vi "Test_Prepare_Checks_Caraya.vi"(8 "error in":errorcluster) -> (0 "error out":errorcluster)   [LabVIEW 2026]
doc: "Caraya tests of Prepare Checks: comparison text to enum, group contents kept, unknown comparison refused."
uses:
  <vilib>/addons/_JKI Toolkits/Caraya/classes/Test/Test.lvclass
  <vilib>/addons/_JKI Toolkits/Caraya/classes/Assert/Assert.lvclass
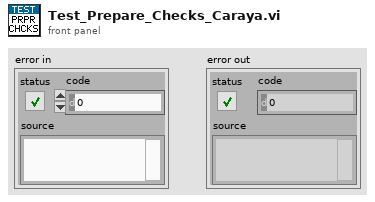
[diagram p1: front panel]
types:
  T1 = cluster{"di_high":cluster{"and":string[], "or":string[]}, "di_low":cluster{"and":string[], "or":string[]}, "misc_high":cluster{"and":string[], "or":string[]}, "misc_low":cluster{"and":string[], "or":string[]}, "t0_high":cluster{"and":cluster{"name":string, "min":dbl, "max":dbl}[], "or":cluster{"name":string, "min":dbl, "max":dbl}[]}, "t0_low":cluster{"and":cluster{"name":string, "min":dbl, "max":dbl}[], "or":cluster{"name":string, "min":dbl, "max":dbl}[]}, "misc_compare":cluster{"name":string, "compare_with":string, "comparison":string, "tolerance":dbl}[]}
  T2 = cluster{"di_high":cluster{"and_list":string[], "or_list":string[]}, "di_low":cluster{"and_list":string[], "or_list":string[]}, "misc_high":cluster{"and_list":string[], "or_list":string[]}, "misc_low":cluster{"and_list":string[], "or_list":string[]}, "t0_high":cluster{"and_list":cluster{"name":string, "min":dbl, "max":dbl}[], "or_list":cluster{"name":string, "min":dbl, "max":dbl}[]}, "t0_low":cluster{"and_list":cluster{"name":string, "min":dbl, "max":dbl}[], "or_list":cluster{"name":string, "min":dbl, "max":dbl}[]}, "misc_compare":cluster{"name":string, "compare_with":string, "comparison":enum16{"EQ", "NE", "GT", "GE", "LT", "LE"}, "tolerance":dbl}[]}
  T3 = cluster{"and_list":cluster{"name":string, "min":dbl, "max":dbl}[], "or_list":cluster{"name":string, "min":dbl, "max":dbl}[]}
  T4 = cluster{"name":string, "compare_with":string, "comparison":enum16{"EQ", "NE", "GT", "GE", "LT", "LE"}, "tolerance":dbl}[]
  T5 = cluster{"name":string, "compare_with":string, "comparison":enum16{"EQ", "NE", "GT", "GE", "LT", "LE"}, "tolerance":dbl}
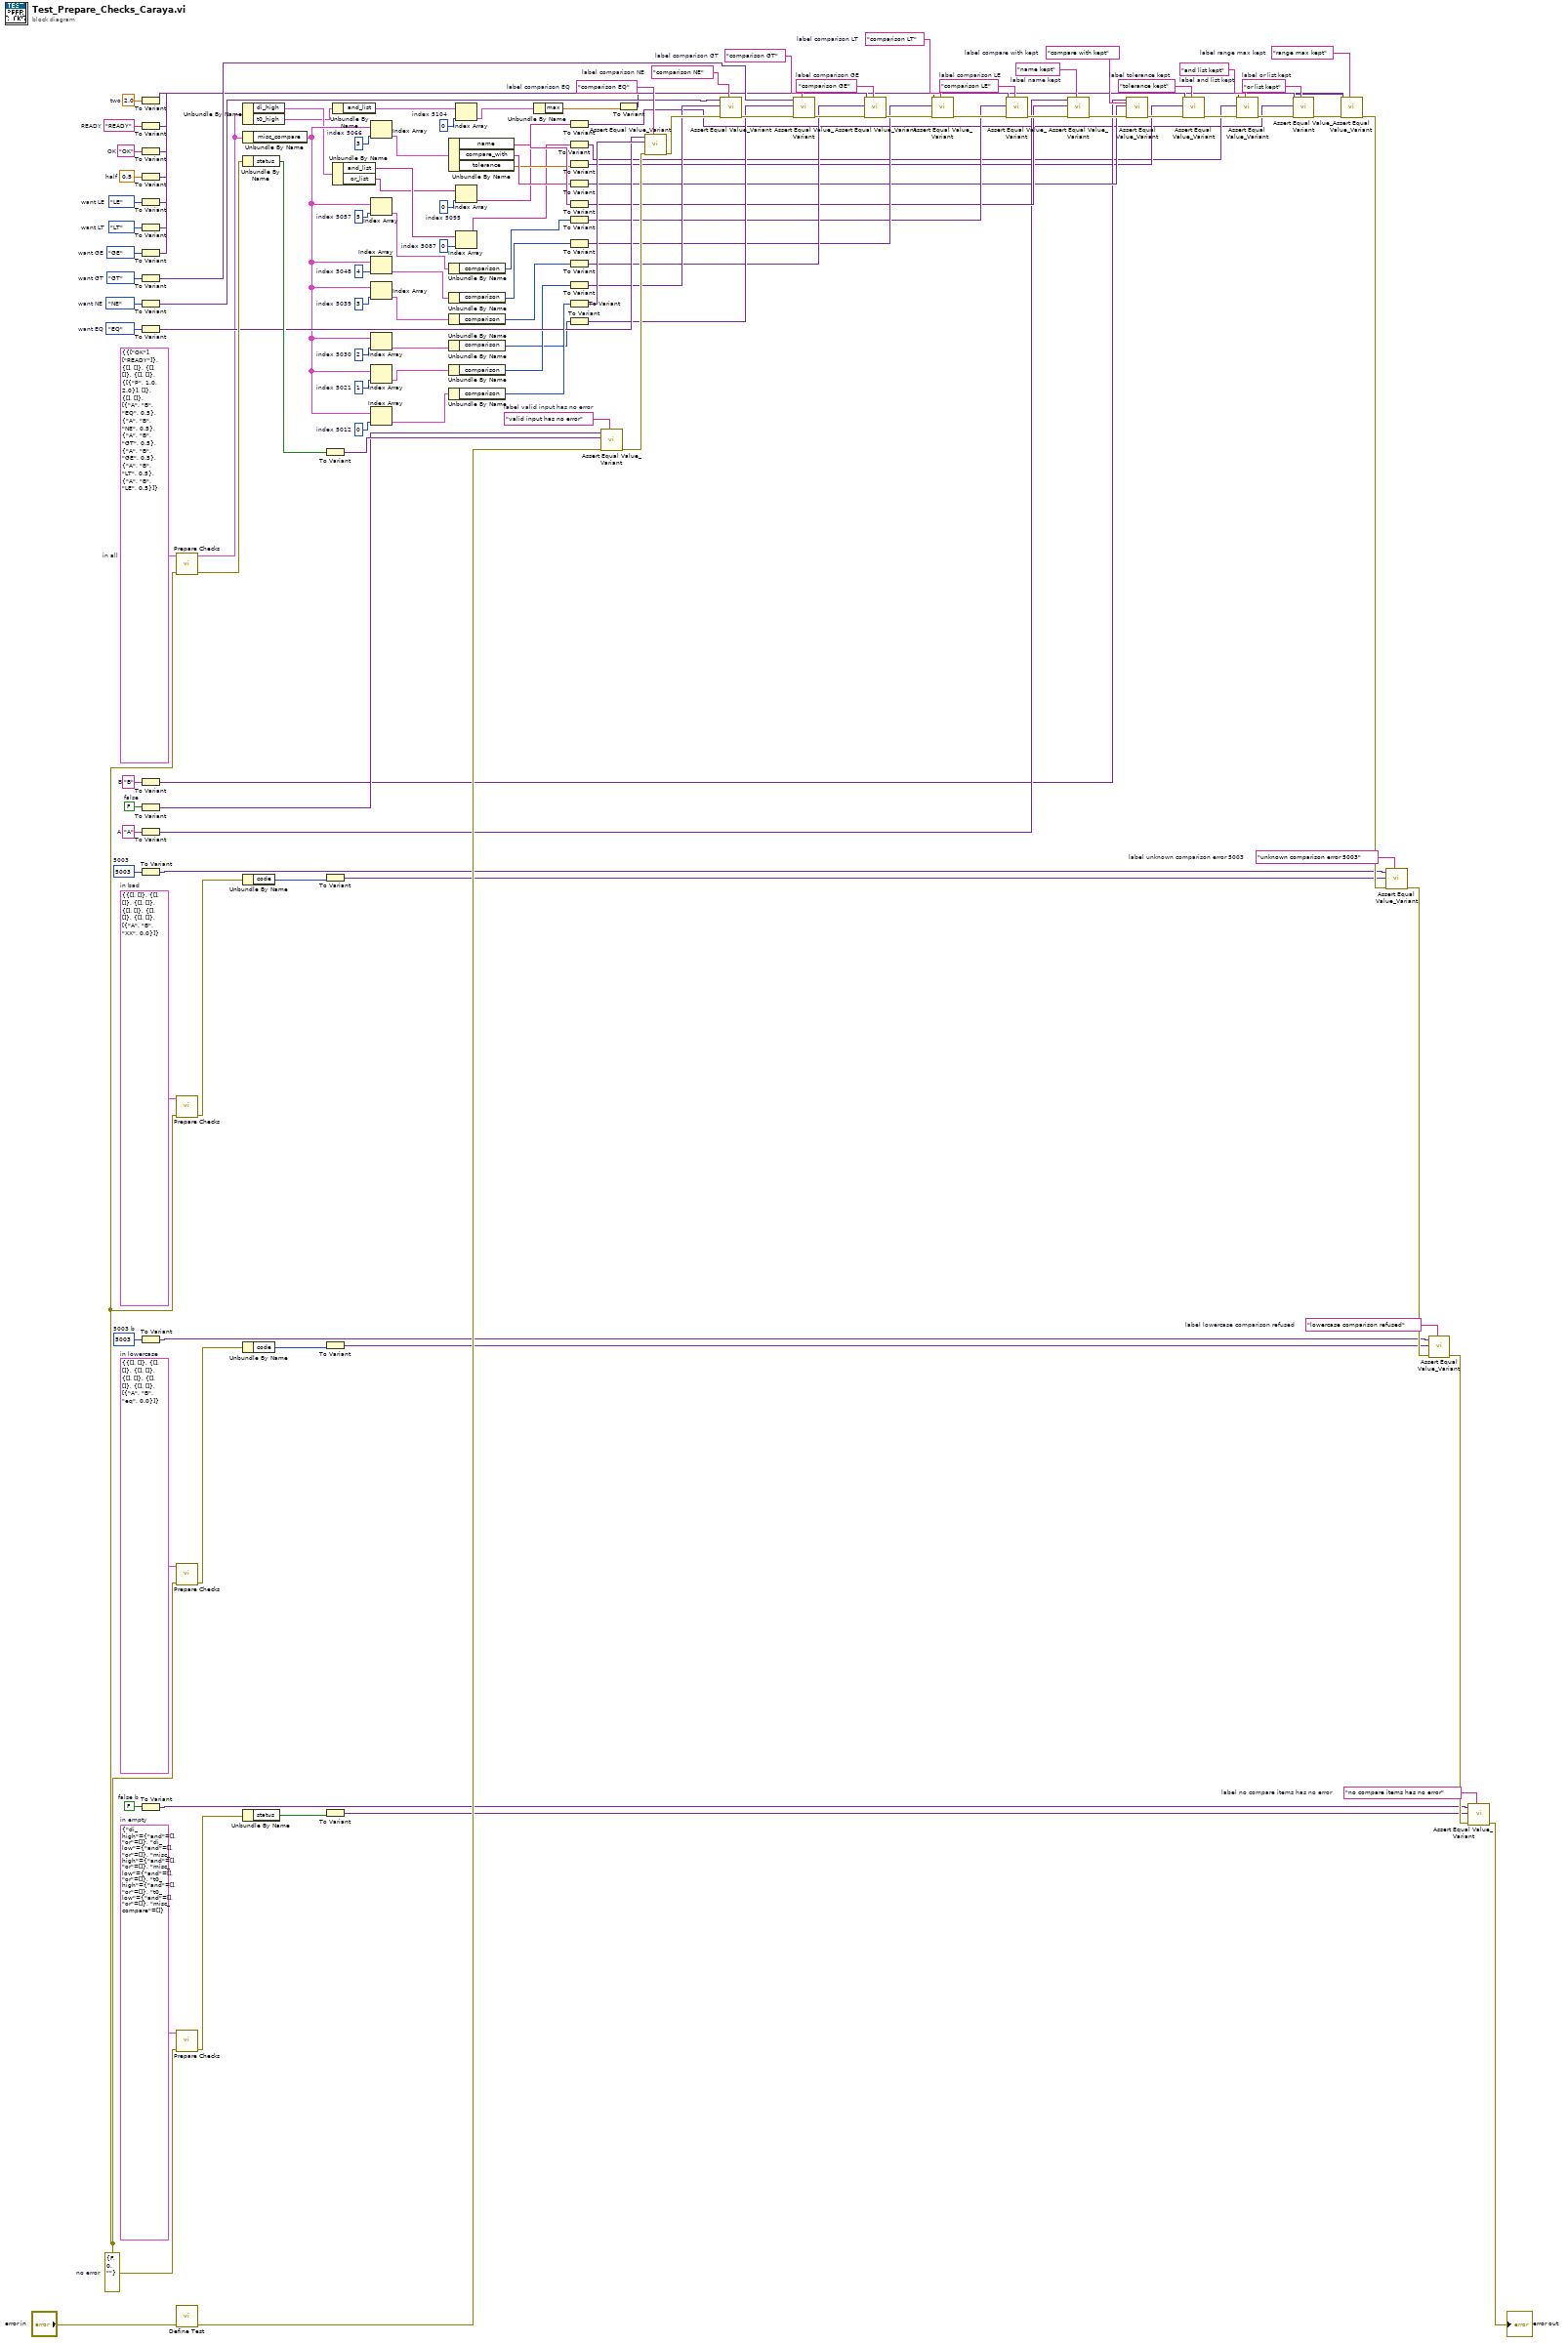
[diagram p0: block diagram]
diagram:
  w5 = "no compare items has no error"  # label no compare items has no error
  w6 = FALSE  # false b
  w10 = T1 {"di_high"={"and"=[], "or"=[]}, "di_low"={"and"=[], "or"=[]}, "misc_high"={"and"=[], "or"=[]}, "misc_low"={"and"=[], "or"=[]}, "t0_high"={"and"=[], "or"=[]}, "t0_low"={"and"=[], "or"=[]}, "misc_compare"=[]}  # in empty
  w14 = "lowercase comparison refused"  # label lowercase comparison refused
  w15 = 5003  # 5003 b
  w18 = T1 {"di_high"={"and"=[], "or"=[]}, "di_low"={"and"=[], "or"=[]}, "misc_high"={"and"=[], "or"=[]}, "misc_low"={"and"=[], "or"=[]}, "t0_high"={"and"=[], "or"=[]}, "t0_low"={"and"=[], "or"=[]}, "misc_compare"=[{"name"="A", "compare_with"="B", "comparison"="eq", "tolerance"=0.0}]}  # in lowercase
  w22 = "unknown comparison error 5003"  # label unknown comparison error 5003
  w23 = 5003  # 5003
  w26 = T1 {"di_high"={"and"=[], "or"=[]}, "di_low"={"and"=[], "or"=[]}, "misc_high"={"and"=[], "or"=[]}, "misc_low"={"and"=[], "or"=[]}, "t0_high"={"and"=[], "or"=[]}, "t0_low"={"and"=[], "or"=[]}, "misc_compare"=[{"name"="A", "compare_with"="B", "comparison"="XX", "tolerance"=0.0}]}  # in bad
  w30 = "range max kept"  # label range max kept
  w31 = 2.0  # two
  w34 = 0  # index 5104
  w40 = "or list kept"  # label or list kept
  w41 = "READY"  # READY
  w43 = 0  # index 5095
  w48 = "and list kept"  # label and list kept
  w49 = "OK"  # OK
  w51 = 0  # index 5087
  w58 = "tolerance kept"  # label tolerance kept
  w59 = 0.5  # half
  w64 = "compare with kept"  # label compare with kept
  w65 = "B"  # B
  w70 = "name kept"  # label name kept
  w71 = "A"  # A
  w74 = 3  # index 5066
  w79 = "comparison LE"  # label comparison LE
  w80 = enum16{"EQ", "NE", "GT", "GE", "LT", "LE"}."LE"  # want LE
  w83 = 5  # index 5057
  w87 = "comparison LT"  # label comparison LT
  w88 = enum16{"EQ", "NE", "GT", "GE", "LT", "LE"}."LT"  # want LT
  w91 = 4  # index 5048
  w95 = "comparison GE"  # label comparison GE
  w96 = enum16{"EQ", "NE", "GT", "GE", "LT", "LE"}."GE"  # want GE
  w99 = 3  # index 5039
  w103 = "comparison GT"  # label comparison GT
  w104 = enum16{"EQ", "NE", "GT", "GE", "LT", "LE"}."GT"  # want GT
  w107 = 2  # index 5030
  w111 = "comparison NE"  # label comparison NE
  w112 = enum16{"EQ", "NE", "GT", "GE", "LT", "LE"}."NE"  # want NE
  w115 = 1  # index 5021
  w119 = "comparison EQ"  # label comparison EQ
  w120 = enum16{"EQ", "NE", "GT", "GE", "LT", "LE"}."EQ"  # want EQ
  w123 = 0  # index 5012
  w127 = "valid input has no error"  # label valid input has no error
  w128 = FALSE  # false
  w131 = T1 {"di_high"={"and"=["OK"], "or"=["READY"]}, "di_low"={"and"=[], "or"=[]}, "misc_high"={"and"=[], "or"=[]}, "misc_low"={"and"=[], "or"=[]}, "t0_high"={"and"=[{"name"="P", "min"=1.0, "max"=2.0}], "or"=[]}, "t0_low"={"and"=[], "or"=[]}, "misc_compare"=[{"name"="A", "compare_with"="B", "comparison"="EQ", "tolerance"=0.5}, {"name"="A", "compare_with"="B", "comparison"="NE", "tolerance"=0.5}, {"name"="A", "compare_with"="B", "comparison"="GT", "tolerance"=0.5}, {"name"="A", "compare_with"="B", "comparison"="GE", "tolerance"=0.5}, {"name"="A", "compare_with"="B", "comparison"="LT", "tolerance"=0.5}, {"name"="A", "compare_with"="B", "comparison"="LE", "tolerance"=0.5}]}  # in all
  w9 = errorcluster {"status"=FALSE, "code"=0, "source"=""}  # no error
  n1 = To Variant(anything=w31) -> (Variant=w27:variant)
  n2 = To Variant(anything=w41) -> (Variant=w37:variant)
  n3 = To Variant(anything=w49) -> (Variant=w45:variant)
  n4 = To Variant(anything=w59) -> (Variant=w55:variant)
  n5 = To Variant(anything=w80) -> (Variant=w76:variant)
  n6 = To Variant(anything=w88) -> (Variant=w84:variant)
  n7 = To Variant(anything=w96) -> (Variant=w92:variant)
  n8 = To Variant(anything=w104) -> (Variant=w100:variant)
  n9 = To Variant(anything=w112) -> (Variant=w108:variant)
  n10 = To Variant(anything=w120) -> (Variant=w116:variant)
  n11 = To Variant(anything=w65) -> (Variant=w61:variant)
  n12 = To Variant(anything=w128) -> (Variant=w124:variant)
  n13 = To Variant(anything=w71) -> (Variant=w67:variant)
  n14 = To Variant(anything=w23) -> (Variant=w19:variant)
  n15 = To Variant(anything=w15) -> (Variant=w11:variant)
  n16 = To Variant(anything=w6) -> (Variant=w2:variant)
  n17 = call "Prepare Checks.vi"("error in"=w9, "checks"=w131) -> ("error out"=w130:errorcluster, "Prepared Checks"=w54:T2)  [unwired: 8 in]
  n18 = call "Prepare Checks.vi"("error in"=w9, "checks"=w26) -> ("error out"=w25:errorcluster)  [unwired: 8 in, 1 out]
  n19 = call "Prepare Checks.vi"("error in"=w9, "checks"=w18) -> ("error out"=w17:errorcluster)  [unwired: 8 in, 1 out]
  n20 = call "Prepare Checks.vi"("error in"=w9, "checks"=w10) -> ("error out"=w8:errorcluster)  [unwired: 8 in, 1 out]
  n21 = call <vilib>:"Define Test.vi"("error in (no error)"="error in") -> ("error out"=w126:errorcluster)  [unwired: 9 in, 1 out]
  n22 = Unbundle By Name(w54) -> ("di_high"=w53:cluster{"and_list":string[], "or_list":string[]}, "t0_high"=w36:T3)
  n23 = Unbundle By Name(w54) -> ("misc_compare"=w75:T4)
  n24 = Unbundle By Name(w130) -> ("status"=w129:bool)
  n25 = Unbundle By Name(w25) -> ("code"=w24:i32)
  n26 = Unbundle By Name(w17) -> ("code"=w16:i32)
  n27 = Unbundle By Name(w8) -> ("status"=w7:bool)
  n28 = To Variant(anything=w129) -> (Variant=w125:variant)
  n29 = To Variant(anything=w24) -> (Variant=w20:variant)
  n30 = To Variant(anything=w16) -> (Variant=w12:variant)
  n31 = To Variant(anything=w7) -> (Variant=w3:variant)
  n32 = Unbundle By Name(w36) -> ("and_list"=w35:cluster{"name":string, "min":dbl, "max":dbl}[])
  n33 = Unbundle By Name(w53) -> ("and_list"=w52:string[], "or_list"=w44:string[])
  n34 = Index Array(array=w75, index=w74) -> (element=w73:T5)
  n35 = Index Array(array=w75, index=w83) -> (element=w82:T5)
  n36 = Index Array(array=w75, index=w91) -> (element=w90:T5)
  n37 = Index Array(array=w75, index=w99) -> (element=w98:T5)
  n38 = Index Array(array=w75, index=w107) -> (element=w106:T5)
  n39 = Index Array(array=w75, index=w115) -> (element=w114:T5)
  n40 = Index Array(array=w75, index=w123) -> (element=w122:T5)
  n41 = Unbundle By Name(w73) -> ("name"=w72:string, "compare_with"=w66:string, "tolerance"=w60:dbl)
  n42 = Unbundle By Name(w82) -> ("comparison"=w81:enum16{"EQ", "NE", "GT", "GE", "LT", "LE"})
  n43 = Unbundle By Name(w90) -> ("comparison"=w89:enum16{"EQ", "NE", "GT", "GE", "LT", "LE"})
  n44 = Unbundle By Name(w98) -> ("comparison"=w97:enum16{"EQ", "NE", "GT", "GE", "LT", "LE"})
  n45 = Unbundle By Name(w106) -> ("comparison"=w105:enum16{"EQ", "NE", "GT", "GE", "LT", "LE"})
  n46 = Unbundle By Name(w114) -> ("comparison"=w113:enum16{"EQ", "NE", "GT", "GE", "LT", "LE"})
  n47 = Unbundle By Name(w122) -> ("comparison"=w121:enum16{"EQ", "NE", "GT", "GE", "LT", "LE"})
  n48 = Index Array(array=w35, index=w34) -> (element=w33:cluster{"name":string, "min":dbl, "max":dbl})
  n49 = Index Array(array=w44, index=w43) -> (element=w42:string)
  n50 = Index Array(array=w52, index=w51) -> (element=w50:string)
  n51 = Unbundle By Name(w33) -> ("max"=w32:dbl)
  n52 = To Variant(anything=w42) -> (Variant=w38:variant)
  n53 = To Variant(anything=w50) -> (Variant=w46:variant)
  n54 = To Variant(anything=w60) -> (Variant=w56:variant)
  n55 = To Variant(anything=w66) -> (Variant=w62:variant)
  n56 = To Variant(anything=w72) -> (Variant=w68:variant)
  n57 = To Variant(anything=w81) -> (Variant=w77:variant)
  n58 = To Variant(anything=w89) -> (Variant=w85:variant)
  n59 = To Variant(anything=w97) -> (Variant=w93:variant)
  n60 = To Variant(anything=w113) -> (Variant=w109:variant)
  n61 = To Variant(anything=w121) -> (Variant=w117:variant)
  n62 = To Variant(anything=w105) -> (Variant=w101:variant)
  n63 = call <vilib>:"Assert Equal Value_Variant.vi"("Label"=w127, "error in (no error)"=w126, "Actual"=w125, "Expected"=w124) -> ("error out"=w118:errorcluster)  [unwired: 6 in, 1 out]
  n64 = To Variant(anything=w32) -> (Variant=w28:variant)
  n65 = call <vilib>:"Assert Equal Value_Variant.vi"("Label"=w119, "error in (no error)"=w118, "Actual"=w117, "Expected"=w116) -> ("error out"=w110:errorcluster)  [unwired: 6 in, 1 out]
  n66 = call <vilib>:"Assert Equal Value_Variant.vi"("Label"=w111, "error in (no error)"=w110, "Actual"=w109, "Expected"=w108) -> ("error out"=w102:errorcluster)  [unwired: 6 in, 1 out]
  n67 = call <vilib>:"Assert Equal Value_Variant.vi"("Label"=w103, "error in (no error)"=w102, "Actual"=w101, "Expected"=w100) -> ("error out"=w94:errorcluster)  [unwired: 6 in, 1 out]
  n68 = call <vilib>:"Assert Equal Value_Variant.vi"("Label"=w95, "error in (no error)"=w94, "Actual"=w93, "Expected"=w92) -> ("error out"=w86:errorcluster)  [unwired: 6 in, 1 out]
  n69 = call <vilib>:"Assert Equal Value_Variant.vi"("Label"=w87, "error in (no error)"=w86, "Actual"=w85, "Expected"=w84) -> ("error out"=w78:errorcluster)  [unwired: 6 in, 1 out]
  n70 = call <vilib>:"Assert Equal Value_Variant.vi"("Label"=w79, "error in (no error)"=w78, "Actual"=w77, "Expected"=w76) -> ("error out"=w69:errorcluster)  [unwired: 6 in, 1 out]
  n71 = call <vilib>:"Assert Equal Value_Variant.vi"("Label"=w70, "error in (no error)"=w69, "Actual"=w68, "Expected"=w67) -> ("error out"=w63:errorcluster)  [unwired: 6 in, 1 out]
  n72 = call <vilib>:"Assert Equal Value_Variant.vi"("Label"=w64, "error in (no error)"=w63, "Actual"=w62, "Expected"=w61) -> ("error out"=w57:errorcluster)  [unwired: 6 in, 1 out]
  n73 = call <vilib>:"Assert Equal Value_Variant.vi"("Label"=w58, "error in (no error)"=w57, "Actual"=w56, "Expected"=w55) -> ("error out"=w47:errorcluster)  [unwired: 6 in, 1 out]
  n74 = call <vilib>:"Assert Equal Value_Variant.vi"("Label"=w48, "error in (no error)"=w47, "Actual"=w46, "Expected"=w45) -> ("error out"=w39:errorcluster)  [unwired: 6 in, 1 out]
  n75 = call <vilib>:"Assert Equal Value_Variant.vi"("Label"=w40, "error in (no error)"=w39, "Actual"=w38, "Expected"=w37) -> ("error out"=w29:errorcluster)  [unwired: 6 in, 1 out]
  n76 = call <vilib>:"Assert Equal Value_Variant.vi"("Label"=w30, "error in (no error)"=w29, "Actual"=w28, "Expected"=w27) -> ("error out"=w21:errorcluster)  [unwired: 6 in, 1 out]
  n77 = call <vilib>:"Assert Equal Value_Variant.vi"("Label"=w22, "error in (no error)"=w21, "Actual"=w20, "Expected"=w19) -> ("error out"=w13:errorcluster)  [unwired: 6 in, 1 out]
  n78 = call <vilib>:"Assert Equal Value_Variant.vi"("Label"=w14, "error in (no error)"=w13, "Actual"=w12, "Expected"=w11) -> ("error out"=w4:errorcluster)  [unwired: 6 in, 1 out]
  n79 = call <vilib>:"Assert Equal Value_Variant.vi"("Label"=w5, "error in (no error)"=w4, "Actual"=w3, "Expected"=w2) -> ("error out"=→"error out":errorcluster)  [unwired: 6 in, 1 out]
